vi "Update Enum Setter.vi"(7 "RPC Message Name":string, 8 "error in (no error)":errorcluster, 10 "Message Getter in":refnum<vi>, 11 "RPC Messages Folder (ProjectItem) in":refnum<vi>) -> (0 "error out":errorcluster, 2 "Message Getter out":refnum<vi>, 3 "RPC Messages Folder (ProjectItem) out":refnum<vi>)   [LabVIEW 2019, in "gRPC Template Creation Utility.lvlib"]
uses:
  gRPC Template Creation Utility.lvlib
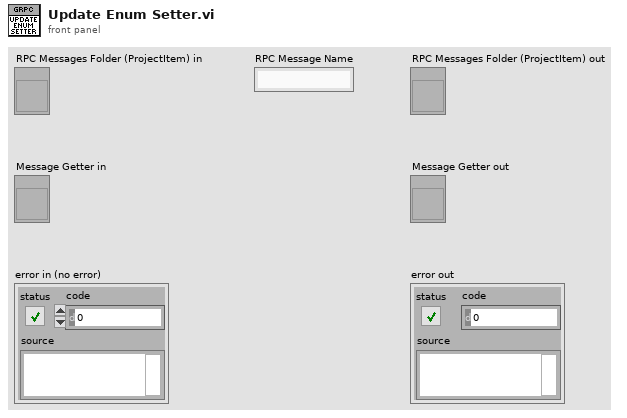
[diagram p1: front panel]
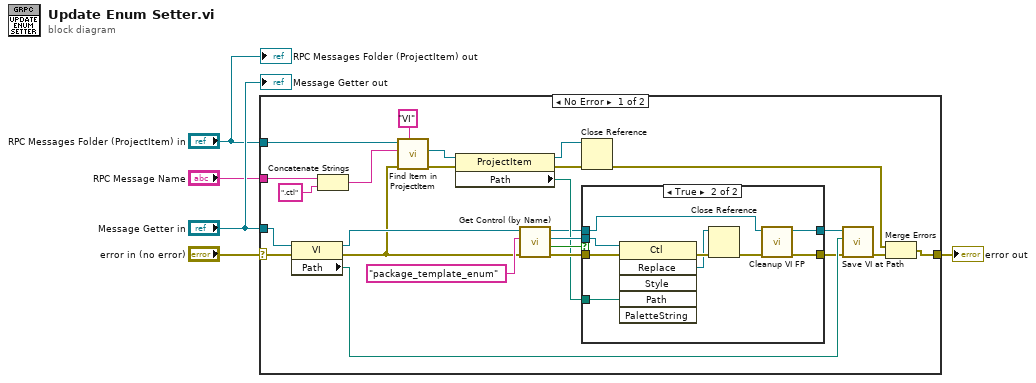
[diagram p0: block diagram]
diagram:
  n1 = case shown="No Error" "error in (no error)" {
    selector: "error in (no error)" -> [w12 w42]
    tunnel: "Message Getter in" -> [w29 _]
    tunnel: [w28 w42] -> w4
    tunnel: "RPC Message Name" -> [w19 _]
    tunnel: "RPC Messages Folder (ProjectItem) in" -> [w17 _]
    frame No Error {
      n2 = property class="VI"(reference=w29, error in=w12) -> (reference out=w13:refnum<vi>, error out=w9:errorcluster, "Path"=w30:path)
      n3 = Concatenate Strings(w19, ".ctl" ("string")) -> (w21:string)
      n4 = call "Find Item in ProjectItem.vi"("Item Type"="VI", "error in (no error)"=w9, "Name"=w21, "ProjectItem in"=w17) -> ("error out"=w23:errorcluster, "Item Refnum out"=w22:refnum<vi>)  [unwired: 4 in, 2 out]
      n5 = property class="ProjectItem"(reference=w22, error in=w23) -> (reference out=w24:refnum<vi>, error out=w25:errorcluster, "Path"=w10:path)
      n6 = call "Get Control (by Name).vi"("error in (no error)"=w9, "Control Label"="package_template_enum" ("name/order"), "Owner VI in"=w13) -> ("error out"=w15:errorcluster, "Found ?"=w16:bool, "Control Refnum"=w14:refnum<vi>, "Owner VI out"=w8:refnum<vi>)  [unwired: 5 in]
      n7 = Close Reference(reference=w24, error in (no error)=w25) -> (error out=w27:errorcluster)
      n8 = case shown="True" w16 {
        tunnel: [w32 w35] -> w6
        tunnel: w14 -> [_ w39]
        tunnel: w15 -> [w32 w38]
        tunnel: w10 -> [_ w37]
        tunnel: w8 -> [w31 w34]
        tunnel: [w31 w33] -> w7
        frame False {
        }
        frame True {
          n9 = invoke class="Ctl" method="Replace"(reference=w39, error in=w38, "Path"=w37) -> (error out=w41:errorcluster, "Replace"=w40:refnum<vi>)  [unwired: 3 in, 4 out]
          n10 = Close Reference(reference=w40, error in (no error)=w41) -> (error out=w36:errorcluster)
          n11 = call "Cleanup VI FP.vi"("error in"=w36, "vi in"=w34) -> ("error out"=w35:errorcluster, "vi out"=w33:refnum<vi>)  [unwired: 8 in]
        }
      }
      n12 = call "Save VI at Path.vi"("error in (no error)"=w6, "Path"=w30, "VI in"=w7) -> ("error out"=w26:errorcluster)  [unwired: 6 in, 2 out]
      n13 = Merge Errors(w27, w26) -> (w28:errorcluster)
    }
    frame Error {
    }
  }
  "error out" <- w4
  "RPC Messages Folder (ProjectItem) out" <- "RPC Messages Folder (ProjectItem) in"
  "Message Getter out" <- "Message Getter in"
